vi "Create Index Array.vi"   [LabVIEW 2012, in "Scripting Tools.lvlib"]
uses:
  Scripting Tools.lvlib
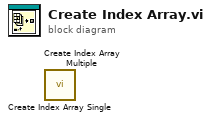
[diagram p0: block diagram]
diagram:
  n1 = call "Create Index Array Single.vi"() -> ()  [unwired: 9 in, 3 out]
  n2 = call "Create Index Array Multiple.vi"() -> ()  [unwired: 9 in, 3 out]
